vi "carrier_enum.vi"() -> ()   [LabVIEW 2019]
doc: "Carrier for typedef probe"
panel:
  in  "Probe Enum":enum16{"ALPHA", "BETA", "GAMMA"}(ring)
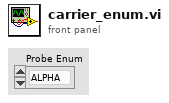
[diagram p1: front panel]
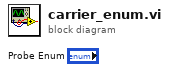
[diagram p0: block diagram]
diagram:
